vi "Open VIRef to Compile.vi"(8 "error in (no error)":errorcluster, 9 "Contains Compiled Code":bool=TRUE, 10 "milliseconds to wait":u32, 11 "dup path":path) -> (0 "error out":errorcluster)   [LabVIEW 2017]
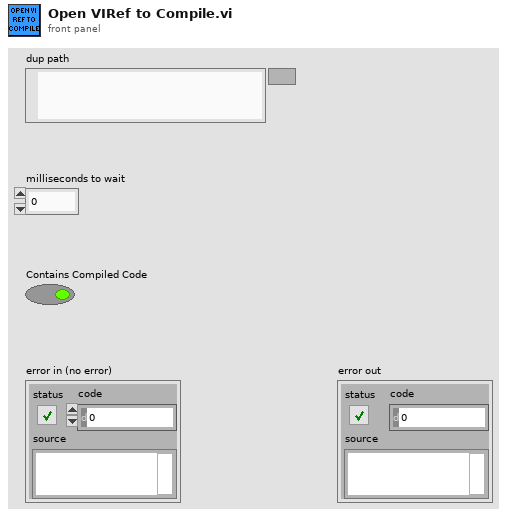
[diagram p1: front panel]
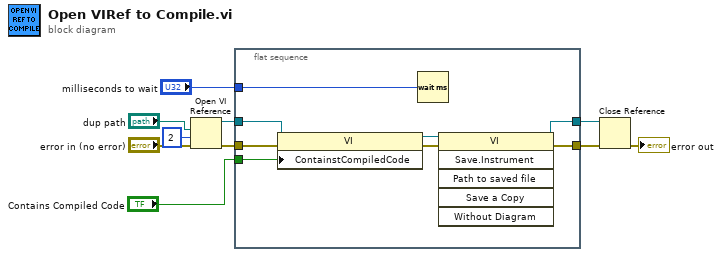
[diagram p0: block diagram]
diagram:
  n1 = Open VI Reference(vi path="dup path", options=2, error in (no error)="error in (no error)") -> (vi reference=w6:refnum<vi>, error out=w2:errorcluster)  [unwired: 3 in]
  n2 = flat-sequence {
    tunnel: w2 -> [w18]
    tunnel: [w17] -> w3
    tunnel: [w16] -> w5
    tunnel: w6 -> [w14]
    tunnel: "milliseconds to wait" -> [w12]
    tunnel: "Contains Compiled Code" -> [w11]
    frame #0 {
      n3 = property class="VI"(reference=w14, error in=w18, "ContainstCompiledCode"=w11) -> (reference out=w13:refnum<vi>, error out=w15:errorcluster)
      n4 = Wait (ms)(milliseconds to wait=w12) -> ()  [unwired: 1 out]
      n5 = invoke class="VI" method="Save.Instrument"(reference=w13, error in=w15) -> (reference out=w16:refnum<vi>, error out=w17:errorcluster)  [unwired: 4 in, 4 out]
    }
  }
  n6 = Close Reference(reference=w5, error in (no error)=w3) -> (error out=→"error out":errorcluster)
